vi "RemoteVI Check Format Duration.vi"() -> (4 "labels":string[](array[string]), 6 "expected":string[](array[string]), 8 "actual":string[](array[string]), 10 "failures":i32)   [LabVIEW 2020]
doc: "Test support, generated by tests/caraya/build.py from tests/vectors/status.json (durations) - do not edit. Calls RemoteVI Format Duration.vi once per vector: the text is compared as the string it is. Outputs, one element per vector: labels (the vector's name), expected (rendered from the vector), actual (the VI's result rendered the same way), and failures, the number of vectors whose expected and actual differ."
uses:
  source/RemoteVI.lvlib
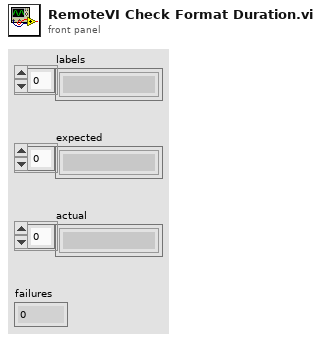
[diagram p1: front panel]
types:
  T1 = cluster{"name":string, "seconds":dbl, "expect":string}[]
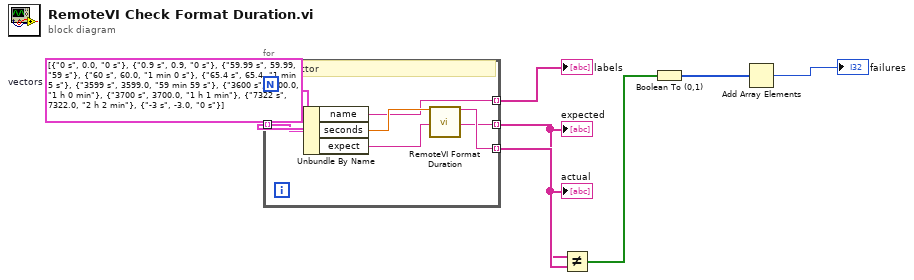
[diagram p0: block diagram]
diagram:
  w1 = T1 [{"name"="0 s", "seconds"=0.0, "expect"="0 s"}, {"name"="0.9 s", "seconds"=0.9, "expect"="0 s"}, {"name"="59.99 s", "seconds"=59.99, "expect"="59 s"}, {"name"="60 s", "seconds"=60.0, "expect"="1 min 0 s"}, {"name"="65.4 s", "seconds"=65.4, "expect"="1 min 5 s"}, {"name"="3599 s", "seconds"=3599.0, "expect"="59 min 59 s"}, {"name"="3600 s", "seconds"=3600.0, "expect"="1 h 0 min"}, {"name"="3700 s", "seconds"=3700.0, "expect"="1 h 1 min"}, {"name"="7322 s", "seconds"=7322.0, "expect"="2 h 2 min"}, {"name"="-3 s", "seconds"=-3.0, "expect"="0 s"}]  # vectors
  n1 = for {
    tunnel: w1 -> [w8] mode=indexing
    tunnel: [w9] -> w2 mode=indexing
    tunnel: [w11] -> w3 mode=indexing
    tunnel: [w12] -> w4 mode=indexing
    # "One vector"
    n2 = Unbundle By Name(w8) -> ("name"=w9:string, "seconds"=w10:dbl, "expect"=w11:string)
    n3 = call "RemoteVI Format Duration.vi"("seconds"=w10) -> ("text"=w12:string)  [unwired: 14 in]
  }
  "labels" <- w2
  "expected" <- w3
  "actual" <- w4
  n4 = Not Equal?(x=w3, y=w4) -> (x != y?=w5:bool[])
  n5 = Boolean To (0,1)(Boolean=w5) -> (0, 1=w6:i16[])
  n6 = Add Array Elements(numeric array=w6) -> (sum=→"failures":i16)
